vi "SP - get subpanel ref.vi"(8 "error in (no error)":errorcluster, 11 "subpanel":string) -> (0 "error out":errorcluster, 1 "subpanel ref":refnum<vi>, 2 "subpanel found ?":bool, 3 "subpanel VI ref":refnum<vi>)   [LabVIEW 2020, in "ui-testing.lvlib"]
uses:
  ui-testing.lvlib
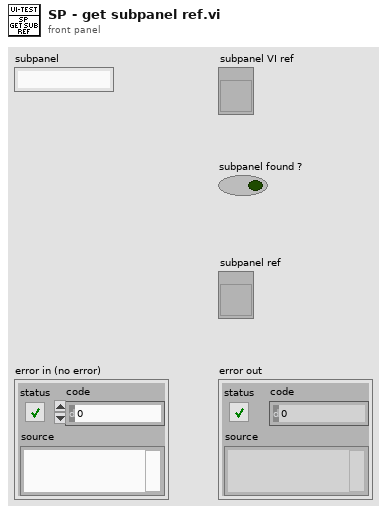
[diagram p1: front panel]
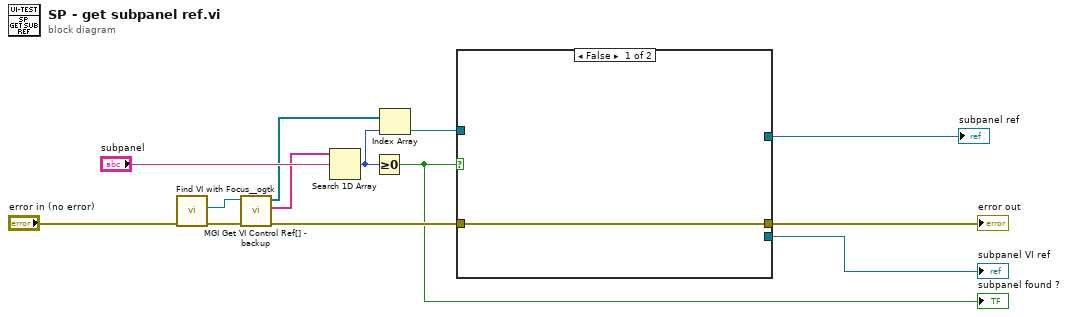
[diagram p0: block diagram]
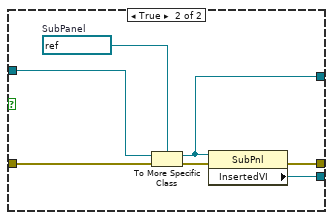
[diagram p2: hidden frame]
diagram:
  n1 = call <userlib>:"Find VI with Focus__ogtk.vi"("error in"="error in (no error)") -> ("error out"=w9:errorcluster, "VI with Focus"=w6:refnum<vi>)  [unwired: 6 in, 3 out]
  n2 = call "MGI Get VI Control Ref[] - backup.vi"("error in"=w9, "VI (Caller)"=w6) -> ("error out"=w10:errorcluster, "Control Label Chain[i]"=w4:string[], "Control[i]"=w3:refnum<vi>[])  [unwired: 6 in, 1 out]
  n3 = Search 1D Array(1D array=w4, element="subpanel") -> (index of element=w5:i32)  [unwired: 1 in]
  n4 = Greater Or Equal To 0?(x=w5) -> (x >= 0?=w1:bool)
  "subpanel found ?" <- w1
  n5 = Index Array(array=w3, index=w5) -> (element=w7:refnum<vi>)
  n6 = case shown="False" w1 {
    tunnel: [w14 w21] -> w13
    tunnel: [_ w20] -> w12
    tunnel: [_ w18] -> w11
    tunnel: w10 -> [w14 w16]
    tunnel: w7 -> [_ w15]
    frame False {
    }
    frame True {
      w17 = refnum<vi> refnum  # SubPanel
      n7 = To More Specific Class(target class=w17, reference=w15, error in=w16) -> (specific class reference=w18:refnum<vi>, error out=w19:errorcluster)
      n8 = property class="SubPnl"(reference=w18, error in=w19) -> (error out=w21:errorcluster, "InsertedVI"=w20:refnum<vi>)  [unwired: 1 out]
    }
  }
  "error out" <- w13
  "subpanel VI ref" <- w12
  "subpanel ref" <- w11
